vi "Wait.vi"(8 "에러 상수 입력":errorcluster caption="에러 상수", 11 "대기 시간 (ms)":u32) -> (0 "에러 상수 출력":errorcluster caption="에러 상수")   [LabVIEW 2023, in "Turn Table and Mast.lvlib" / "CO3000.lvclass"]
uses:
  CO3000.lvclass
  CO3000.lvclass/CO3000.ctl
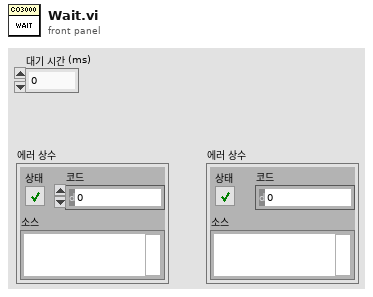
[diagram p1: front panel]
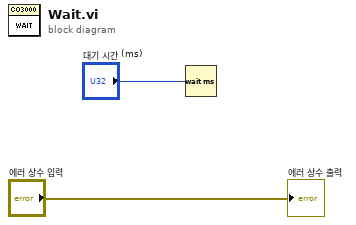
[diagram p0: block diagram]
diagram:
  n1 = Wait (ms)(milliseconds to wait="대기 시간 (ms)") -> ()  [unwired: 1 out]
  "에러 상수 출력" <- "에러 상수 입력"
